vi "Client.vi"() -> ()   [LabVIEW 2020]
uses:
  source/PV Data/NT Scalar/NT Scalar.lvclass
  C:/Users/eyw68381/source/repos/pvaccess-labview/labview/source/PV Data/NT Base/NT Base.lvclass
  C:/Users/eyw68381/source/repos/pvaccess-labview/labview/source/PV Data/Base/Base.lvclass
  C:/Users/eyw68381/source/repos/pvaccess-labview/labview/source/PV Data/Base Interface/Base Interface.lvclass
  C:/Users/eyw68381/source/repos/pvaccess-labview/labview/source/PV Data/Has Alarm/Has Alarm.lvclass
  C:/Users/eyw68381/source/repos/pvaccess-labview/labview/source/PV Data/Has Time Stamp/Has Time Stamp.lvclass
  C:/Users/eyw68381/source/repos/pvaccess-labview/labview/source/PV Data/NT Scalar/NT Scalar.lvclass
  source/PV Data/NT Scalar (Numeric)/NT Scalar (Numeric).lvclass
  C:/Users/eyw68381/source/repos/pvaccess-labview/labview/source/PV Data/Has Alarm Limits/Has Alarm Limits.lvclass
  C:/Users/eyw68381/source/repos/pvaccess-labview/labview/source/PV Data/Has Control Limits/Has Control Limits.lvclass
  C:/Users/eyw68381/source/repos/pvaccess-labview/labview/source/PV Data/NT Scalar (Numeric)/NT Scalar (Numeric).lvclass
  source/Client/Client/Client.lvclass
  source/Client/Client/Get - NT Scalar (Numeric).vi
  source/Client/Client/Get - NT Scalar.vi
  source/PV Data/Type Code.ctl
  source/PV Data/PV Data.lvlib
panel:
  out "Precision":i32
  out "type code":T1
  out "value":variant
  in  "PV name":string="DEV:FLOAT64"
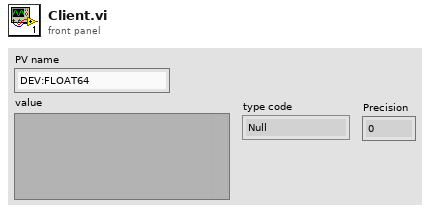
[diagram p1: front panel]
types:
  T1 = typedef "PV Access.lvlib/PV Data.lvlib/Type Code.ctl" = enum8{"Null", "Bool", "BoolA", "Int8", "Int8A", "Int16", "Int16A", "Int32", "Int32A", "Int64", "Int64A", "UInt8", "UInt8A", "UInt16", "UInt16A", "UInt32", "UInt32A", "UInt64", "UInt64A", "Float32", "Float32A", "Float64", "Float64A", "String", "StringA", "Struct", "StructA", "Union", "UnionA", "Any", "AnyA"}
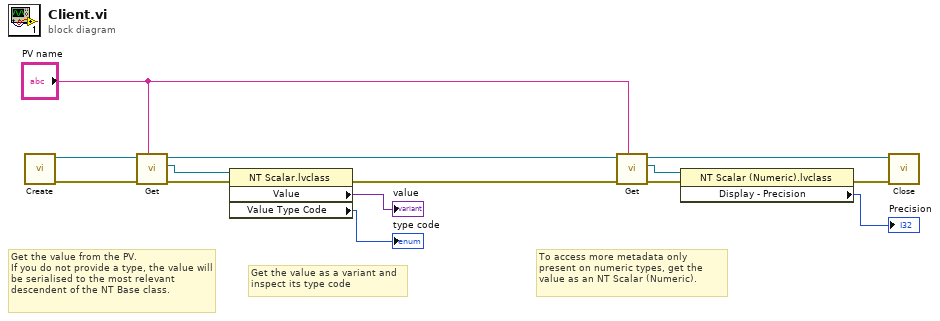
[diagram p0: block diagram]
diagram:
  # "To access more metadata only present on numeric types, get the value as an NT Scalar (Numeric)."
  # "Get the value as a variant and inspect its type code"
  # "Get the value from the PV.\nIf you do not provide a type, the value will be serialised to the most relevant descendent of the NT Base class."
  n1 = call "Create.vi"() -> ("error out"=w13:errorcluster, "Client out"=w14:refnum<class "Client.lvclass">)  [unwired: 10 in]
  n2 = call-poly "Get.vi"("PV name"="PV name", "error in (no error)"=w13, "Client in"=w14) -> ("error out"=w12:errorcluster, "value"=w11:refnum<class "NT Scalar.lvclass">, "Client out"=w8:refnum<class "Client.lvclass">)  [unwired: 5 in, 1 out]
  n3 = property class="NT Scalar.lvclass"(reference=w11, error in=w12) -> (error out=w6:errorcluster, "Value"=→"value":variant, "Value Type Code"=→"type code":T1)  [unwired: 1 out]
  n4 = call-poly "Get.vi"("PV name"="PV name", "error in (no error)"=w6, "Client in"=w8) -> ("error out"=w5:errorcluster, "value"=w3:refnum<class "NT Scalar (Numeric).lvclass">, "Client out"=w2:refnum<class "Client.lvclass">)  [unwired: 5 in, 1 out]
  n5 = property class="NT Scalar (Numeric).lvclass"(reference=w3, error in=w5) -> (error out=w4:errorcluster, "Display - Precision"=→"Precision":i32)  [unwired: 1 out]
  n6 = call "Close.vi"("error in (no error)"=w4, "Client in"=w2) -> ()  [unwired: 9 in, 1 out]
